vi "matlab_radar_plot.vi"(3 "error in":errorcluster, 4 "radar data cube":string, 5 "Radar Sample":T1, 6 "Radar configuration":string="{\n  \"type\": \"Radar\",\n   \"gpu_number\":0,\n  \"listen_port\": 8301,\n  \"send_radar_cube\":false,\n  \"paint_targets\": false,\n  \"target_paint_lifetime\": 0.5,\n  \"location\": {\n    \"x\": 250.0,\n    \"y\": 0.0,\n    \"z\": 50.0\n  },\n  \"rotation\": {\n    \"pitch\": 0.0,\n    \"yaw\": 0.0,\n    \"roll\": 0.0\n  },\n  \"num_samples_per_sweep\":345,\n  \"fs\": 50000000,\n  \"fc\": 77000000000.0,\n  \"num_sweeps\": 32,\n  \"sweep_time\" : 0.0000069,\n  \"bandwidth\" : 172500000,\n  \"max_targets\": 250,\n  \"elements\": 8,\n  \"transmitter\": {\n    \"peak_power\": 5.0,\n    \"aperture\": 0.000859,\n    \"gain\": 13.50\n  },\n  \"receiver\": {\n    \"aperture\": 0.000798,\n    \"nf\": 10.0,\n    \"noise_temp\": 290.0,\n    \"nb\": 74000000.0,\n    \"gain\": 10.0\n  },\n  \"sbr\": {\n    \"long_range_scan_distance\": 150.0,\n    \"short_range_scan_distance\": 60.0,\n    \"long_range_fov\": 20.0,\n    \"short_range_fov\": 60.0,\n    \"elevation_fov\": 10.0,\n    \"rescan_density\": 20.0,\n    \"debug_frustum\": false,\n    \"debug_scan\": false,\n    \"debug_rescan\": false\n  }\n}") -> (0 "error out":errorcluster)   [LabVIEW 2019]
doc: "Process radar data cube and run a Matlab script to plot Radar cube data."
uses:
  controls/radarSample.ctl
  controls/RadarTrack.ctl
panel:
  out "Success":dbl
  out "Size":dbl
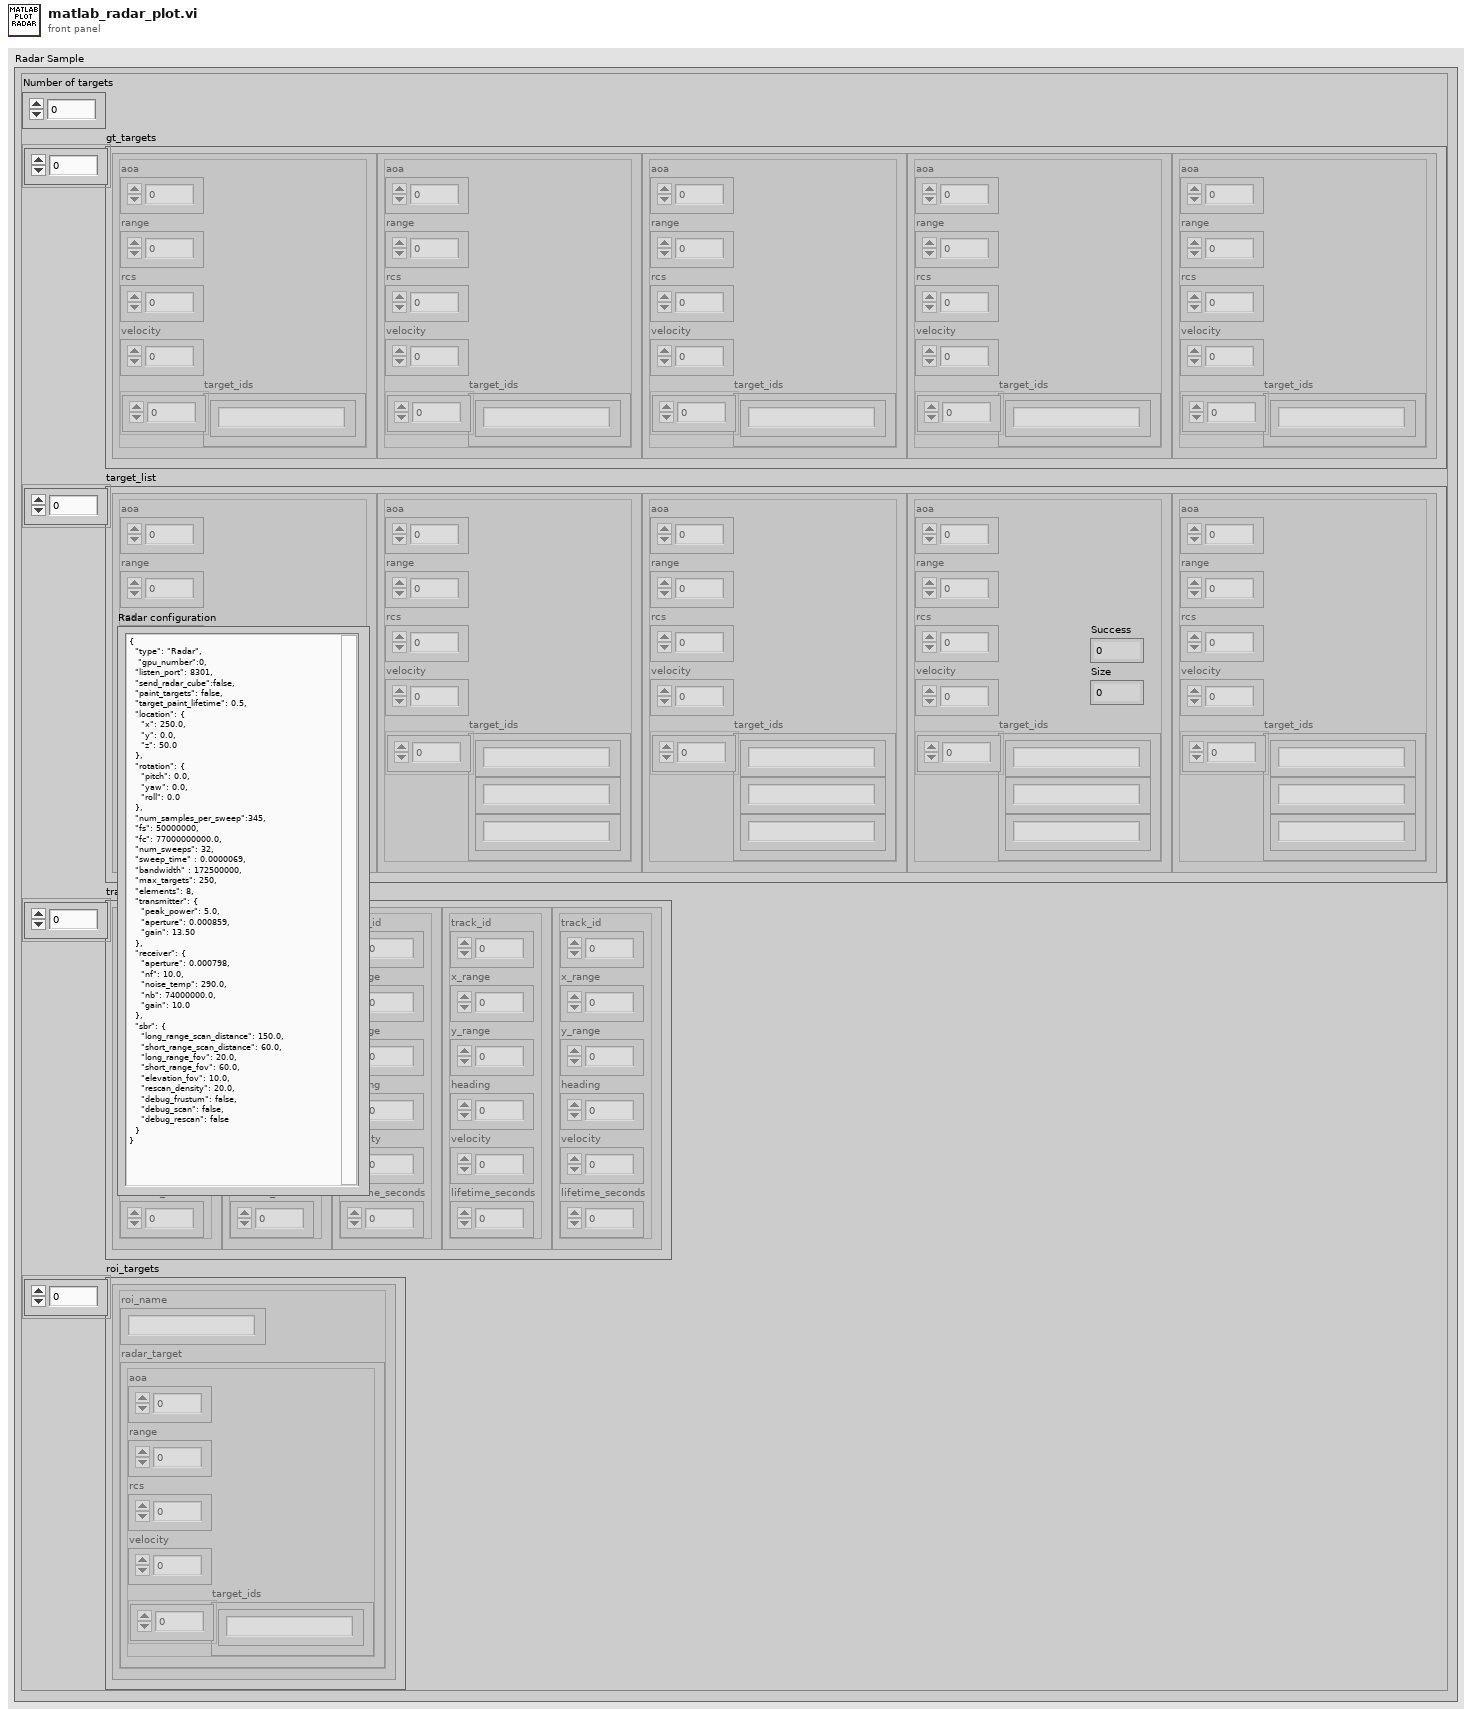
[diagram p1: front panel]
types:
  T1 = typedef "radarSample.ctl" = cluster{"Number of targets":i32, "gt_targets":cluster{"aoa":sgl, "range":sgl, "rcs":sgl, "velocity":sgl, "target_ids":string[]}[], "target_list":cluster{"aoa":sgl, "range":sgl, "rcs":sgl, "velocity":sgl, "target_ids":string[]}[], "tracks":T2[], "roi_targets":cluster{"roi_name":string, "radar_target":cluster{"aoa":sgl, "range":sgl, "rcs":sgl, "velocity":sgl, "target_ids":string[]}}[]}
  T2 = typedef "RadarTrack.ctl" = cluster{"track_id":u64, "x_range":sgl, "y_range":sgl, "heading":sgl, "velocity":sgl, "lifetime_seconds":sgl}
  T3 = cluster{"aoa":sgl, "range":sgl, "rcs":sgl, "velocity":sgl, "target_ids":string[]}[]
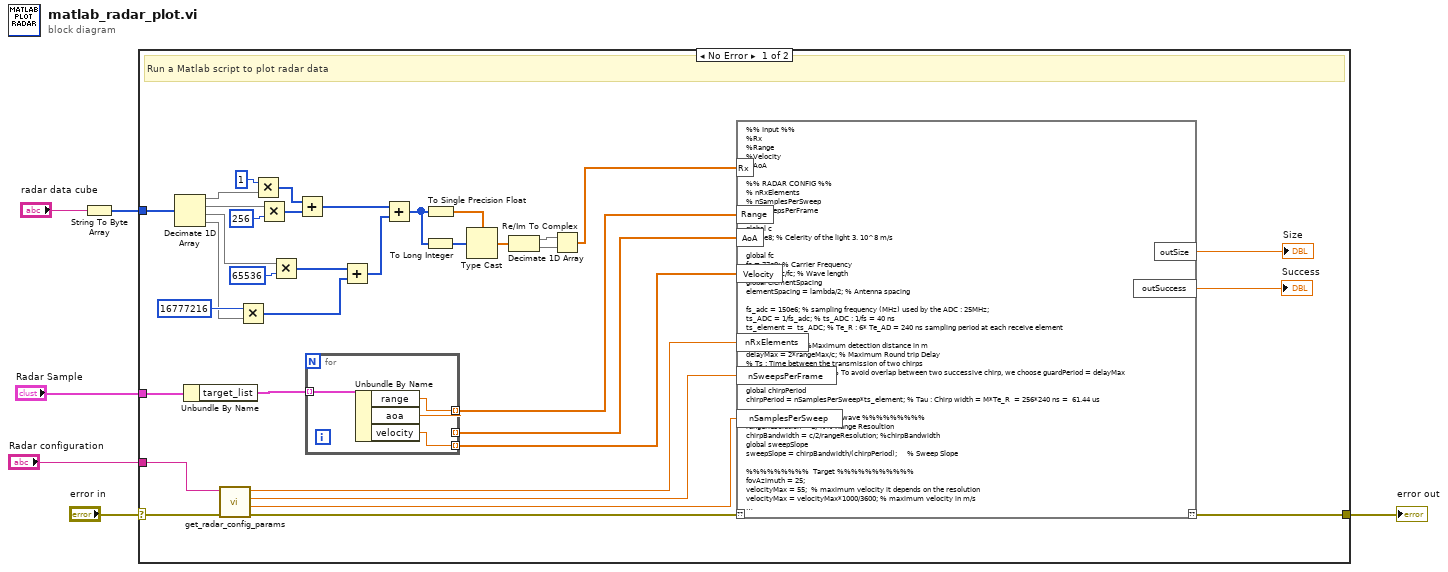
[diagram p0: block diagram]
diagram:
  n1 = String To Byte Array(string="radar data cube") -> (unsigned byte array=w4:u8[])
  n2 = case shown="No Error" "error in" {
    selector: "error in" -> [w11 w47]
    tunnel: "Radar Sample" -> [w21 _]
    tunnel: w4 -> [w32 _]
    tunnel: "Radar configuration" -> [w13 _]
    tunnel: [w12 w47] -> w1
    frame No Error {
      # "Run a Matlab script to plot radar data"
      n3 = Decimate 1D Array(w32) -> (w30:u8[], w42:u8[], w39:u8[], w37:u8[])
      n4 = Unbundle By Name(w21) -> ("target_list"=w20:T3)
      n5 = call "get_radar_config_params.vi"("error in"=w11, "Radar configuration"=w13) -> ("error out"=w10:errorcluster, "num_samples_per_sweep"=w7:dbl, "num_sweeps"=w8:dbl, "elements"=w9:dbl)  [unwired: 2 in]
      n6 = Multiply(x=16777216, y=w37) -> (x*y=w35:i32[])
      n7 = Multiply(x=1, y=w30) -> (x*y=w31:i32[])
      n8 = Multiply(x=w42, y=256) -> (x*y=w36:i32[])
      n9 = Multiply(x=w39, y=65536) -> (x*y=w34:i32[])
      n10 = Add(x=w31, y=w36) -> (x+y=w28:i32[])
      n11 = for {
        tunnel: w20 -> [w46] mode=indexing
        tunnel: [w45] -> w19 mode=indexing
        tunnel: [w44] -> w18 mode=indexing
        tunnel: [w43] -> w17 mode=indexing
        n12 = Unbundle By Name(w46) -> ("range"=w45:sgl, "aoa"=w44:sgl, "velocity"=w43:sgl)
      }
      n13 = Add(x=w34, y=w35) -> (x+y=w33:i32[])
      n14 = Add(x=w28, y=w33) -> (x+y=w26:i32[])
      n15 = To Long Integer(number=w26) -> (32bit integer=w27:i32[])
      n16 = To Single Precision Float(number=w26) -> (single precision float=w25:sgl[])
      n17 = Type Cast(type=w25, x=w27) -> (*(type *) &x=w24:sgl[])
      n18 = Decimate 1D Array(w24) -> (w23:sgl[], w22:sgl[])
      n19 = Re/Im To Complex(1:w22, 2:w23) -> (0:w16:csg[])
      n20 = script code="%% Input %%\n%Rx\n%Range\n%Velocity\n%AoA\n\n%% RADAR CONFIG %%\n% nRxElements\n% nSamplesPerSweep\n% nSweepsPerFrame\n\nglobal c\nc = 3e8; % Celerity of the light 3. 10^8 m/s\n\nglobal fc\nfc = 77e9; % Carrier Frequency\nlambda = c/fc; % Wave length\nglobal elementSpacing\nelementSpacing = lambda/2; % Antenna spacing\n\nfs_adc = 150e6; % sampling frequency (MHz) used by the ADC : 25MHz;\nts_ADC = 1/fs_adc; % ts_ADC : 1/fs = 40 ns\nts_element =  ts_ADC; % Te_R : 6* Te_AD = 240 ns sampling period at each receive element\n\nrangeMax = 125; %Maximum detection distance in m\ndelayMax = 2*rangeMax/c; % Maximum Round trip Delay\n% Ts : Time between the transmission of two chirps\nguardPeriod = delayMax; % To avoid overlap between two successive chirp, we choose guardPeriod = delayMax\n\nglobal chirpPeriod\nchirpPeriod = nSamplesPerSweep*ts_element; % Tau : Chirp width = M*Te_R  = 256*240 ns =  61.44 us\n\n%%%%%%%%%% FMCW wave %%%%%%%%%\nrangeResolution = 1; %% Range Resoultion\nchirpBandwidth = c/2/rangeResolution; %chirpBandwidth\nglobal sweepSlope\nsweepSlope = chirpBandwidth/(chirpPeriod);     % Sweep Slope\n\n%%%%%%%%%  Target %%%%%%%%%%%\nfovAzimuth = 25;\nvelocityMax = 55;  % maximum velocity it depends on the resolution\nvelocityMax = velocityMax*1000/3600; % maximum velocity in m/s\n\nglobal fs_sim;\nfs_sim = 150*1e6; % System Simulation sampling frequency\nglobal ts_sim;\nts_sim = 1/fs_sim; % Simulation system sampling period\nn_decimation = fix(fs_sim/fs_adc); % Down sampling ratio between the simulation system simulator and the ADC sampling frequency\n\nnFFT = 1024;\nnFFT_Doppler = 1024;\nnFFT_AoA = 1024;\nfs_doppler = 1 / chirpPeriod;\nDelta_f = fs_doppler / nFFT_Doppler / 2;\ndoppler_bin_size = Delta_f * lambda;\n%binSize_aoa = 1; NOT USED\nrange_bin_size = c/ 2 * nSamplesPerSweep / nFFT / fs_adc;\n% Definition of windows used in FFT\n%hann_range = hann(nSamplesPerSweep-100); %window(@gausswin,nSamplesPerSweep,3);\n\nfreq = (0:nFFT/2-1);\ncteRange = 3e8 / 2 * nSamplesPerSweep / 1024 / 150e6 ;\nfreq=freq*cteRange;\n\nsizeRx = length(Rx);\noutSize = sizeRx;\noutSuccess = 0;\n\nif(sizeRx == nSamplesPerSweep * nSweepsPerFrame * nRxElements)\n    outSuccess = 1;    \n\n    data_cube = zeros(nSamplesPerSweep,nSweepsPerFrame,nRxElements);\n    \n    for k=1:nSamplesPerSweep\n        for m=1:nSweepsPerFrame\n            for l=1:nRxElements\n                data_cube(k,m,l)=Rx(k+(l-1)* nSamplesPerSweep +(m-1)* nSamplesPerSweep*nRxElements);\n            end\n        end\n    end\n    \n    t=(0:nSamplesPerSweep-1)*ts_ADC;\n    figure(2)\n    subplot(221)\n    plot(t/1e-6,real(data_cube(:,1,1))/1000);\n    xlabel('Time (\\mu s)'); ylabel('Amplitude (V)');\n    title('Mixed Received Signal at the output of the ADC '); axis tight;\n    \n    grid on\n    %yy=fft2(data_cube(:,:,1).*kron(hann(nSamplesPerSweep),hann(nSweepsPerFrame)'),1024,1024);\n    \n    %yy2=fftshift(yy);\n    %subplot(222); meshRangeDop =  mesh(10*log10(abs(yy2)'/max(max(abs(yy2)))))\n    %direction = [0 0 1];\n    %rotate(meshRangeDop,direction,-90)\n    \n    %title('2D FFT of the received DATA CUBE');\n    %ylabel('For Range Detection', 'Rotation',-17)\n    %xlabel('For Doppler Detection', 'Rotation',12)\n    \n    sweep_idx = 1;\n    sweep = data_cube(:,sweep_idx,1); %reading one sweep\n    %range_FFT = fft(sweep(51:end-50).*hann_range,nFFT); %%% FFT for range detection\n    range_FFT = fft(sweep(51:end-50),nFFT); %%% FFT for range detection\n    range_FFT = range_FFT(1:nFFT/2);\n    range_FFT = abs(range_FFT);\n    \n    zoro=round(Range/cteRange)+1;\n    peaks=0*range_FFT;\n    peaks(zoro)=range_FFT(zoro);\n    \n    subplot(223); plot(freq, 10*log10(range_FFT)-124);\n    hold on;%%%% Plot\n    stem(freq, 10*log10(peaks)-124,'r');\n    xlabel('Equivalent Range (m)')\n    ylabel('PSD of the received Signal ')\n    axis ([0 200 -120 -50])\n    grid on\n    legend('FFT on the Fast Time');\n    hold off\n    \n    subplot(2,2,[2,4]); polarplot(AoA/180*pi,Range,'ro','MarkerSize',6,'MarkerEdgeColor','r',  'MarkerFaceColor','r');\n    ax=gca;\n    ax.ThetaLim = [-30 30];\n    ax.ThetaZeroLocation = 'top';\n    title(' Range vs Angle of Arrival')\n    rticks([0 10 20 30 40 50 60 80 100 120 150 ] )\n    ax.RLim = [0 150];\n    rticklabels({'Range = 0','10',' 20',' 30',' 40', ' 50','60','80','100','120', '150'})\n    ax.ThetaColor = 'blue';\n    ax.RColor = 'red'; %[1 .5 0.3];\n\n    %set(gcf,'units','normalized','outerposition',[0 0 1 0.7])\n    %pause(.1)\n    drawnow\nend"("??"=w10, "Rx"=w16, "Range"=w19, "Velocity"=w17, "AoA"=w18, "nRxElements"=w9, "nSweepsPerFrame"=w8, "nSamplesPerSweep"=w7) -> ("??"=w12:errorcluster, "outSize"=→"Size":dbl, "outSuccess"=→"Success":dbl)
    }
    frame Error {
    }
  }
  "error out" <- w1
